vi "Load Config.vi"(8 "error in (no error)":errorcluster, 11 "PluginGUI in":refnum<class "PluginGUI.lvclass">) -> (0 "error out":errorcluster, 3 "PluginGUI out":refnum<class "PluginGUI.lvclass">)   [LabVIEW 2020, in "VolatusGUI.lvlib" / "PluginGUI.lvclass"]
uses:
  PluginGUI.lvclass
  C:/dev/lv20CE/relink/lv-volatus/Volatus/Module/Module.lvclass
  PluginGUI.lvclass/PluginGUI.ctl
  Volatus/Module/Module.lvclass/Module.ctl
  VolatusConfig/VolatusConfigElement/VolatusConfigElement.lvclass/VolatusConfigElement.ctl
  Volatus/Module/Config.vi
  VolatusConfig/VolatusConfigElement/Element.vi
  VolatusConfig/Task/Task Config.lvclass
  C:/dev/lv20CE/relink/lv-volatus/VolatusConfig/VolatusConfigElement/VolatusConfigElement.lvclass
  Volatus/Module/Module.lvclass
  VolatusConfig/VolatusConfigElement/VolatusConfigElement.lvclass
  lv-cdm/CDM-Config/Config Element/Config Element.lvclass
  Volatus/VolatusAPI/VolatusAPI.lvclass
  C:/dev/lv20CE/relink/lv-volatus/VolatusGUI/PluginGUI/PluginGUI.lvclass
  C:/dev/lv20CE/relink/lv-volatus/VolatusConfig/Task/Task Config.lvclass
  GUI Type.ctl
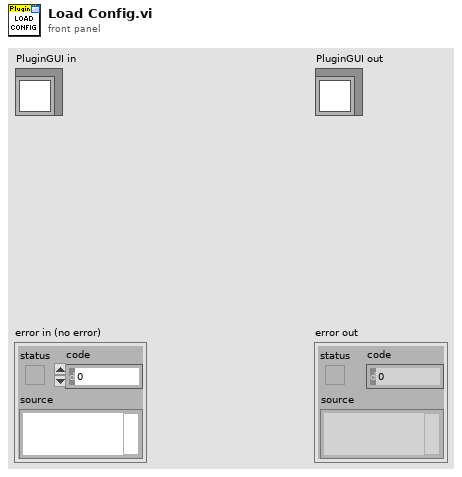
[diagram p1: front panel]
types:
  T1 = typedef "VolatusGUI.lvlib/PluginGUI.lvclass/GUI Type.ctl" = enum16{"Unknown", "Config", "Path", "Ref"}
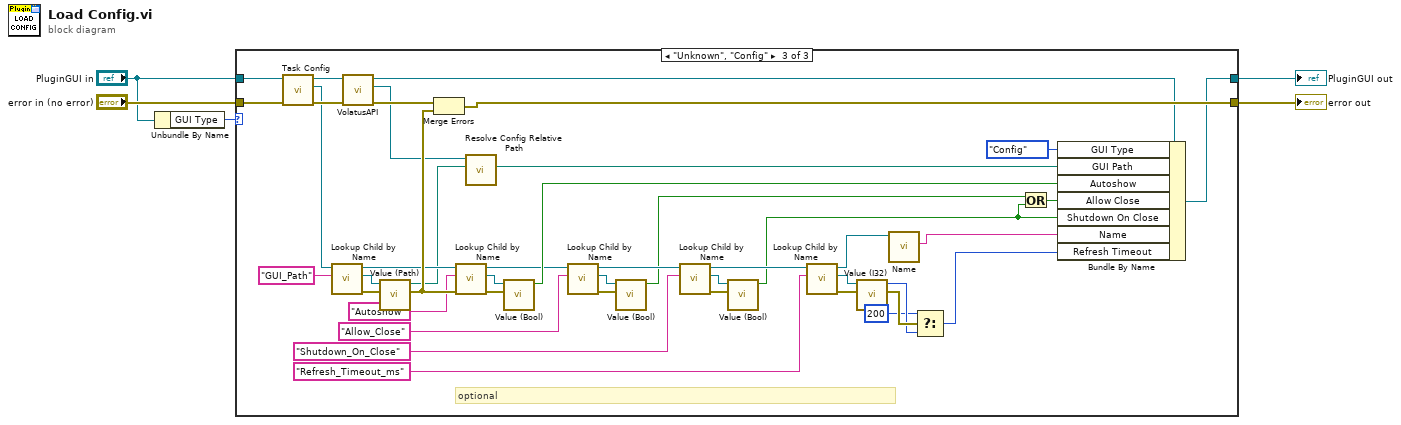
[diagram p0: block diagram]
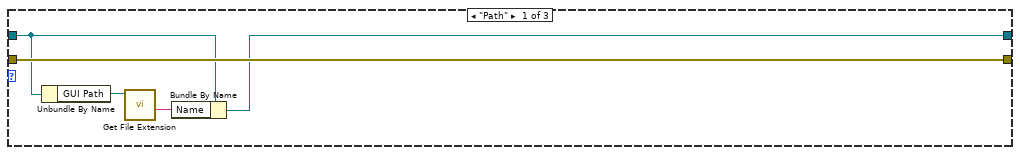
[diagram p2: hidden frame]
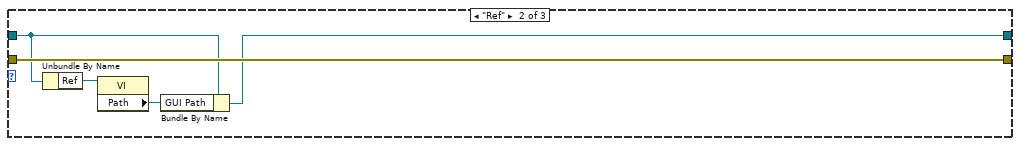
[diagram p3: hidden frame]
diagram:
  n1 = Unbundle By Name("PluginGUI in") -> ("GUI Type"=w1:T1)
  n2 = case shown="\"Unknown\", \"Config\"" w1 {
    tunnel: "error in (no error)" -> [w10 w15 w56]
    tunnel: [w10 w15 w45] -> w4
    tunnel: [w9 w12 w43] -> w3
    tunnel: "PluginGUI in" -> [w7 w14 w19]
    frame "Path" {
      n3 = Unbundle By Name(w7) -> ("GUI Path"=w6:path)
      n4 = call <vilib>:"Get File Extension.vi"("file"=w6) -> ("filename without extension"=w8:string)  [unwired: 6 in, 4 out]
      n5 = Bundle By Name(cluster=w7, "Name"=w8) -> (w9:refnum<class "PluginGUI.lvclass">)
    }
    frame "Ref" {
      n6 = Unbundle By Name(w14) -> ("Ref"=w13:refnum<vi>)
      n7 = property class="VI"(reference=w13) -> ("Path"=w11:path)  [unwired: 1 in, 2 out]
      n8 = Bundle By Name(cluster=w14, "GUI Path"=w11) -> (w12:refnum<class "PluginGUI.lvclass">)
    }
    frame "Unknown", "Config" {
      # "optional"
      n9 = call "Task Config.vi"("error in (no error)"=w56, "Module in"=w19) -> ("error out"=w55:errorcluster, "Task Config"=w54:refnum<class "Task Config.lvclass">, "Module out"=w44:refnum<class "PluginGUI.lvclass">)  [unwired: 7 in]
      n10 = call "Lookup Child by Name.vi"("Child Name"="GUI_Path", "VolatusConfigElement in"=w54) -> ("error out"=w52:errorcluster, "Child"=w51:refnum<class "Config Element.lvclass">, "VolatusConfigElement out"=w50:refnum<class "Task Config.lvclass">)  [unwired: 6 in, 1 out]
      n11 = call "VolatusAPI.vi"("Module in"=w44) -> ("VolatusAPI"=w22:refnum<class "VolatusAPI.lvclass">, "Module out"=w23:refnum<class "PluginGUI.lvclass">)  [unwired: 9 in]
      n12 = call "Value (Path).vi"("error in (no error)"=w52, "Config Element in"=w51) -> ("error out"=w57:errorcluster, "Path Value"=w21:path)  [unwired: 8 in]
      n13 = Merge Errors(w55, w57) -> (w45:errorcluster)
      n14 = call "Lookup Child by Name.vi"("error in (no error)"=w57, "Child Name"="Autoshow", "VolatusConfigElement in"=w50) -> ("error out"=w48:errorcluster, "Child"=w47:refnum<class "Config Element.lvclass">, "VolatusConfigElement out"=w32:refnum<class "Task Config.lvclass">)  [unwired: 5 in, 1 out]
      n15 = call "Resolve Config Relative Path.vi"("Path"=w21, "VolatusAPI in"=w22) -> ("Resolved Path"=w20:path)  [unwired: 7 in, 2 out]
      n16 = call "Value (Bool).vi"("error in (no error)"=w48, "Config Element in"=w47) -> ("Bool Value"=w46:bool)  [unwired: 8 in, 1 out]
      n17 = call "Lookup Child by Name.vi"("Child Name"="Allow_Close", "VolatusConfigElement in"=w32) -> ("error out"=w34:errorcluster, "Child"=w35:refnum<class "Config Element.lvclass">, "VolatusConfigElement out"=w28:refnum<class "Task Config.lvclass">)  [unwired: 6 in, 1 out]
      n18 = call "Value (Bool).vi"("error in (no error)"=w34, "Config Element in"=w35) -> ("Bool Value"=w26:bool)  [unwired: 8 in, 1 out]
      n19 = call "Lookup Child by Name.vi"("Child Name"="Shutdown_On_Close", "VolatusConfigElement in"=w28) -> ("error out"=w30:errorcluster, "Child"=w29:refnum<class "Config Element.lvclass">, "VolatusConfigElement out"=w27:refnum<class "Task Config.lvclass">)  [unwired: 6 in, 1 out]
      n20 = call "Value (Bool).vi"("error in (no error)"=w30, "Config Element in"=w29) -> ("Bool Value"=w25:bool)  [unwired: 8 in, 1 out]
      n21 = call "Lookup Child by Name.vi"("Child Name"="Refresh_Timeout_ms", "VolatusConfigElement in"=w27) -> ("error out"=w41:errorcluster, "Child"=w40:refnum<class "Config Element.lvclass">, "VolatusConfigElement out"=w18:refnum<class "Task Config.lvclass">)  [unwired: 6 in, 1 out]
      n22 = call "Value (I32).vi"("error in (no error)"=w41, "Config Element in"=w40) -> ("error out"=w39:errorcluster, "I32 Value"=w38:i32)  [unwired: 8 in]
      n23 = call "Name.vi"("VolatusConfigElement in"=w18) -> ("Name"=w17:string)  [unwired: 8 in, 2 out]
      n24 = Select(t=200, s=w39, f=w38) -> (s? t:f=w36:i32)
      n25 = Or(x=w26, y=w25) -> (x .or. y?=w31:bool)
      n26 = Bundle By Name(cluster=w23, "GUI Type"=GUI_Type."Config", "GUI Path"=w20, "Autoshow"=w46, "Allow Close"=w31, "Shutdown On Close"=w25, "Name"=w17, "Refresh Timeout"=w36) -> (w43:refnum<class "PluginGUI.lvclass">)
    }
  }
  "error out" <- w4
  "PluginGUI out" <- w3
